vi "detect connected chassis.vi"(8 "error in":errorcluster, 11 "system session in":refnum<k21>) -> (0 "error out":errorcluster, 2 "chassis":T2 {"remote chassis"."product ID" format="%.0x"; "local chassis"."product ID" format="%.0x"}, 3 "system session out":refnum<k21>)   [LabVIEW 2014, in "SMI.lvlib" / "Controller.lvclass"]
uses:
  Controller.lvclass
  Chassis/chassis information.ctl
  <vilib>/nisyscfg/Close (System).vi
  <vilib>/nisyscfg/Close (Filter).vi
  <vilib>/nisyscfg/Close (Resources).vi
  <vilib>/regexp/Match Regular Expression.xnode
  <resource>/objmgr/niflexriosae.rc
  <vilib>/nisyscfg/nisyscfg.lvlib
  <resource>/objmgr/nisysapi.rc
  Chassis/Chassis.lvclass
  SMI.lvlib
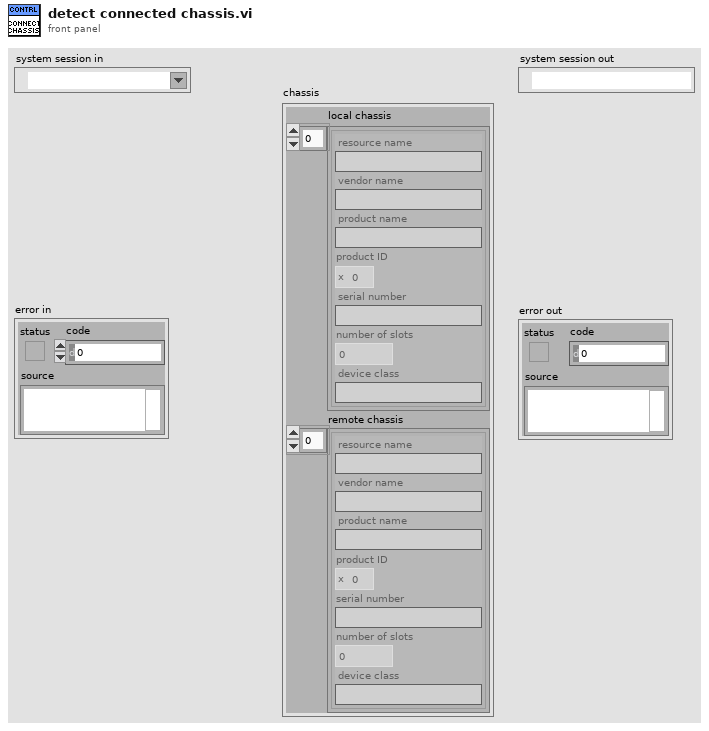
[diagram p1: front panel]
types:
  T1 = typedef "SMI.lvlib/Chassis.lvclass/chassis information.ctl" = cluster{"resource name":string, "vendor name":string, "product name":string, "product ID":u16, "serial number":string, "number of slots":i32, "device class":string}
  T2 = cluster{"local chassis":T1[], "remote chassis":T1[]}
  T3 = cluster{"Local Chassis":T1[], "Remote Chassis":T1[]}
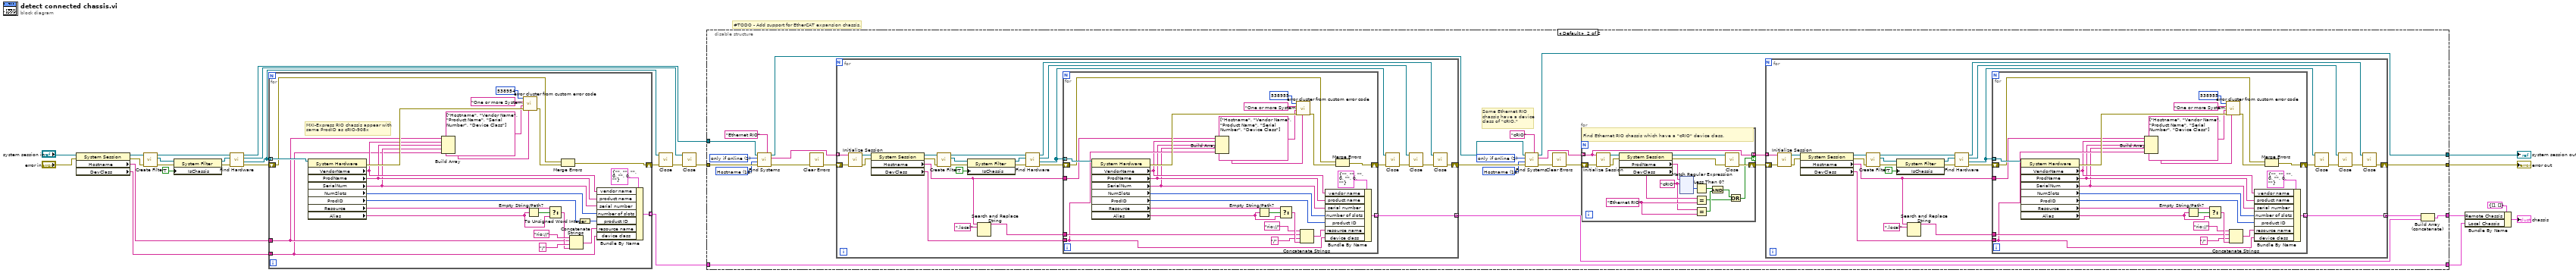
[diagram p0: block diagram]
diagram:
  # "#TODO - Add support for EtherCAT expansion chassis."
  n1 = property class="System Session"(reference="system session in", error in="error in") -> (reference out=w8:refnum<k21>, error out=w7:errorcluster, "Hostname"=w6:string, "DevClass"=w1:string)
  n2 = call <vilib>:"Create Filter.vi"("error in (no error)"=w7, "Session in"=w8) -> ("error out"=w5:errorcluster, "Filter out"=w4:refnum<k20>, "Session out"=w18:refnum<k21>)  [unwired: 7 in]
  n3 = property class="System Filter"(reference=w4, error in=w5, "IsChassis"=TRUE ("Is Chassis")) -> (reference out=w17:refnum<k20>, error out=w16:errorcluster)
  n4 = call <vilib>:"Find Hardware.vi"("error in (no error)"=w16, "Filter in"=w17, "Session in"=w18) -> ("error out"=w15:errorcluster, "Resources out"=w12:refnum<k20>[], "Filter out"=w11:refnum<k20>, "Session out"=w9:refnum<k21>)  [unwired: 5 in]
  n5 = for {
    tunnel: w12 -> [w52] mode=indexing
    shift-right: [w31] -> w13
    shift-left: w15 -> [w33]
    tunnel: [w51] -> w2 mode=indexing
    tunnel: w6 -> [w38]
    tunnel: w1 -> [w34]
    # "MXI-Express RIO chassis appear with\nsame ProdID as cRIO-908x"
    n6 = property class="System Hardware"(reference=w52) -> (error out=w39:errorcluster, "VendorName"=w37:string, "ProdName"=w36:string, "SerialNum"=w35:string, "NumSlots"=w50:i32, "ProdID"=w40:u32, "Resource"=w44:string, "Alias"=w45:string)  [unwired: 1 in, 1 out]
    n7 = Build Array(w38, w37, w36, w35, w34) -> (w29:string[])
    n8 = call "error cluster from custom error code.vi"("string values"=w29, "error in"=w39, "keys"=string[] ["Hostname", "Vendor Name", "Product Name", "Serial Number", "Device Class"], "error message"="One or more System Hardware properties are not available for the target chassis.", "custom error code (0)"=538954 ("error code (0)")) -> ("error out"=w32:errorcluster)  [unwired: 6 in]
    n9 = Empty String/Path?(string/path=w45) -> (empty?=w46:bool)
    n10 = Select(t=w44, s=w46, f=w45) -> (s? t:f=w43:string)
    n11 = Merge Errors(w33, w32) -> (w31:errorcluster)
    n12 = Concatenate Strings("rio://" ("string"), w38, "/" ("string"), w43) -> (w49:string)
    n13 = To Unsigned Word Integer(number=w40) -> (unsigned 16bit integer=w41:u16)
    n14 = Bundle By Name(cluster=T1 {"resource name"="", "vendor name"="", "product name"="", "product ID"=0, "serial number"="", "number of slots"=0, "device class"=""} ("Chassis Information"), "vendor name"=w37, "product name"=w36, "serial number"=w35, "number of slots"=w50, "product ID"=w41, "resource name"=w49, "device class"=w34) -> (w51:T1)
  }
  n15 = call-poly <vilib>:"Close.vi"("error in (no error)"=w13, "Resources in"=w12) -> ("error out"=w14:errorcluster)  [unwired: 9 in]
  n16 = call-poly <vilib>:"Close.vi"("error in (no error)"=w14, "Filter in"=w11) -> ("error out"=w10:errorcluster)  [unwired: 9 in]
  n17 = disable-structure shown="Default" {
    disable-tunnel: w2 -> [w53 w71]
    disable-tunnel: w10 -> [w55 w79]
    disable-tunnel: w9 -> [w54 w78]
    disable-tunnel: [w55 w68] -> w26
    disable-tunnel: [_ w56] -> w21
    disable-tunnel: [w54 w67] -> w23
    disable-tunnel: [w53 w71] -> w20
    frame condition #0 {
      # "Possible CAR: PharLap and VxWorks targets cannot detect Ethernet RIO chassis using Find Systems.vi."
    }
    frame condition #1 (active) {
      w64 = u32 1 items=["none"=0, "only if online"=1, "all"=3] ("Include Cached Results (all)")
      w63 = u32 16 items=["Hostname"=16, "Hostname (IP)"=18, "Hostname (MAC)"=19, "IP"=32, "IP (Hostname)"=33, "IP (MAC)"=35, "MAC"=48, "MAC (Hostname)"=49, "MAC (IP)"=50] ("Output (Hostname and IP)")
      w75 = u32 1 items=["none"=0, "only if online"=1, "all"=3] ("Include Cached Results (all)")
      w76 = u32 16 items=["Hostname"=16, "Hostname (IP)"=18, "Hostname (MAC)"=19, "IP"=32, "IP (Hostname)"=33, "IP (MAC)"=35, "MAC"=48, "MAC (Hostname)"=49, "MAC (IP)"=50] ("Output (Hostname and IP)")
      # "Some Ethernet RIO\nchassis have a device \nclass of \"cRIO.\""
      n18 = call <vilib>:"Find Systems.vi"("Device Class"="Ethernet RIO", "error in (no error)"=w79, "Output (Hostname and IP)"=w76, "Include Cached Results (all)"=w75, "Session in (localhost)"=w78) -> ("error out"=w72:errorcluster, "Detected Systems"=w77:string[], "Session out"=w70:refnum<k21>)  [unwired: 4 in]
      n19 = call <vilib>:"Clear Errors.vi"("error in (no error)"=w72) -> ("error out"=w73:errorcluster)  [unwired: 5 in, 1 out]
      n20 = for {
        shift-right: [w275] -> w69
        shift-left: w73 -> [w286]
        tunnel: [w277] -> w57 mode=concatenating
        tunnel: w77 -> [w273] mode=indexing
        n21 = call <vilib>:"Initialize Session.vi"("error in (no error)"=w286, "Target (localhost)"=w273) -> ("error out"=w270:errorcluster, "Session out"=w272:refnum<k21>)  [unwired: 8 in]
        n22 = property class="System Session"(reference=w272, error in=w270) -> (reference out=w271:refnum<k21>, error out=w269:errorcluster, "Hostname"=w262:string, "DevClass"=w263:string)
        n23 = call <vilib>:"Create Filter.vi"("error in (no error)"=w269, "Session in"=w271) -> ("error out"=w264:errorcluster, "Filter out"=w265:refnum<k20>, "Session out"=w278:refnum<k21>)  [unwired: 7 in]
        n24 = property class="System Filter"(reference=w265, error in=w264, "IsChassis"=TRUE ("Is Chassis")) -> (reference out=w279:refnum<k20>, error out=w280:errorcluster)
        n25 = Search and Replace String(input string=w262, search string=".local") -> (result string=w268:string)  [unwired: 6 in, 3 out]
        n26 = call <vilib>:"Find Hardware.vi"("error in (no error)"=w280, "Filter in"=w279, "Session in"=w278) -> ("error out"=w281:errorcluster, "Resources out"=w284:refnum<k20>[], "Filter out"=w285:refnum<k20>, "Session out"=w276:refnum<k21>)  [unwired: 5 in]
        n27 = for {
          tunnel: w284 -> [w312] mode=indexing
          shift-right: [w296] -> w283
          shift-left: w281 -> [w298]
          tunnel: [w311] -> w277 mode=indexing
          tunnel: w268 -> [w301]
          tunnel: w263 -> [w294]
          tunnel: w262 -> [w295]
          n28 = property class="System Hardware"(reference=w312) -> (error out=w299:errorcluster, "VendorName"=w293:string, "ProdName"=w292:string, "SerialNum"=w291:string, "NumSlots"=w310:i32, "ProdID"=w309:u32, "Resource"=w303:string, "Alias"=w302:string)  [unwired: 1 in, 1 out]
          n29 = Build Array(w295, w293, w292, w291, w294) -> (w288:string[])
          n30 = Empty String/Path?(string/path=w302) -> (empty?=w307:bool)
          n31 = Select(t=w303, s=w307, f=w302) -> (s? t:f=w308:string)
          n32 = call "error cluster from custom error code.vi"("string values"=w288, "error in"=w299, "keys"=string[] ["Hostname", "Vendor Name", "Product Name", "Serial Number", "Device Class"], "error message"="One or more System Hardware properties are not available for the Ethernet RIO remote chassis.", "custom error code (0)"=538955 ("error code (0)")) -> ("error out"=w297:errorcluster)  [unwired: 6 in]
          n33 = Concatenate Strings("rio://" ("string"), w301, "/" ("string"), w308) -> (w304:string)
          n34 = Bundle By Name(cluster=T1 {"resource name"="", "vendor name"="", "product name"="", "product ID"=0, "serial number"="", "number of slots"=0, "device class"=""} ("Chassis Information"), "vendor name"=w293, "product name"=w292, "serial number"=w291, "number of slots"=w310, "product ID"=w309, "resource name"=w304, "device class"=w294) -> (w311:T1)
          n35 = Merge Errors(w298, w297) -> (w296:errorcluster)
        }
        n36 = call-poly <vilib>:"Close.vi"("error in (no error)"=w283, "Resources in"=w284) -> ("error out"=w282:errorcluster)  [unwired: 9 in]
        n37 = call-poly <vilib>:"Close.vi"("error in (no error)"=w282, "Filter in"=w285) -> ("error out"=w274:errorcluster)  [unwired: 9 in]
        n38 = call-poly <vilib>:"Close.vi"("error in (no error)"=w274, "Session in"=w276) -> ("error out"=w275:errorcluster)  [unwired: 9 in]
      }
      n39 = call <vilib>:"Find Systems.vi"("Device Class"="cRIO", "error in (no error)"=w69, "Output (Hostname and IP)"=w63, "Include Cached Results (all)"=w64, "Session in (localhost)"=w70) -> ("error out"=w66:errorcluster, "Detected Systems"=w62:string[], "Session out"=w67:refnum<k21>)  [unwired: 4 in]
      n40 = call <vilib>:"Clear Errors.vi"("error in (no error)"=w66) -> ("error out"=w61:errorcluster)  [unwired: 5 in, 1 out]
      n41 = for {
        tunnel: w62 -> [w94] mode=indexing
        tunnel: [w94] -> w59 mode=indexing if=w80
        shift-right: [w91] -> w60
        shift-left: w61 -> [w93]
        w86 = "cRIO" ("regular expression")
        w89 = "Ethernet RIO" ("y")
        # "Find Ethernet RIO chassis which have a \"cRIO\" device class."
        n42 = call <vilib>:"Initialize Session.vi"("error in (no error)"=w93, "Target (localhost)"=w94) -> ("error out"=w96:errorcluster, "Session out"=w95:refnum<k21>)  [unwired: 8 in]
        n43 = property class="System Session"(reference=w95, error in=w96) -> (reference out=w90:refnum<k21>, error out=w92:errorcluster, "ProdName"=w81:string, "DevClass"=w88:string)
        n44 = xnode "Match Regular Expression"("input string"=w81, "regular expression"=w86) -> ("offset past match"=w87:i32)  [unwired: 4 in, 4 out]
        n45 = Less Than 0?(x=w87) -> (x < 0?=w85:bool)
        n46 = Equal?(x=w88, y=w89) -> (x = y?=w82:bool)
        n47 = Equal?(x=w86, y=w89) -> (x = y?=w84:bool)
        n48 = And(x=w85, y=w84) -> (x .and. y?=w83:bool)
        n49 = call-poly <vilib>:"Close.vi"("error in (no error)"=w92, "Session in"=w90) -> ("error out"=w91:errorcluster)  [unwired: 9 in]
        n50 = Or(x=w83, y=w82) -> (x .or. y?=w80:bool)
      }
      n51 = for {
        shift-right: [w224] -> w68
        shift-left: w60 -> [w235]
        tunnel: [w226] -> w58 mode=concatenating
        tunnel: w59 -> [w222] mode=indexing
        n52 = call <vilib>:"Initialize Session.vi"("error in (no error)"=w235, "Target (localhost)"=w222) -> ("error out"=w219:errorcluster, "Session out"=w221:refnum<k21>)  [unwired: 8 in]
        n53 = property class="System Session"(reference=w221, error in=w219) -> (reference out=w220:refnum<k21>, error out=w218:errorcluster, "Hostname"=w211:string, "DevClass"=w212:string)
        n54 = call <vilib>:"Create Filter.vi"("error in (no error)"=w218, "Session in"=w220) -> ("error out"=w213:errorcluster, "Filter out"=w214:refnum<k20>, "Session out"=w227:refnum<k21>)  [unwired: 7 in]
        n55 = property class="System Filter"(reference=w214, error in=w213, "IsChassis"=TRUE ("Is Chassis")) -> (reference out=w228:refnum<k20>, error out=w229:errorcluster)
        n56 = Search and Replace String(input string=w211, search string=".local") -> (result string=w217:string)  [unwired: 6 in, 3 out]
        n57 = call <vilib>:"Find Hardware.vi"("error in (no error)"=w229, "Filter in"=w228, "Session in"=w227) -> ("error out"=w230:errorcluster, "Resources out"=w233:refnum<k20>[], "Filter out"=w234:refnum<k20>, "Session out"=w225:refnum<k21>)  [unwired: 5 in]
        n58 = for {
          tunnel: w233 -> [w261] mode=indexing
          shift-right: [w245] -> w232
          shift-left: w230 -> [w247]
          tunnel: [w260] -> w226 mode=indexing
          tunnel: w217 -> [w250]
          tunnel: w212 -> [w243]
          tunnel: w211 -> [w244]
          n59 = property class="System Hardware"(reference=w261) -> (error out=w248:errorcluster, "VendorName"=w242:string, "ProdName"=w241:string, "SerialNum"=w240:string, "NumSlots"=w259:i32, "ProdID"=w258:u32, "Resource"=w252:string, "Alias"=w251:string)  [unwired: 1 in, 1 out]
          n60 = Build Array(w244, w242, w241, w240, w243) -> (w237:string[])
          n61 = Empty String/Path?(string/path=w251) -> (empty?=w256:bool)
          n62 = Select(t=w252, s=w256, f=w251) -> (s? t:f=w257:string)
          n63 = call "error cluster from custom error code.vi"("string values"=w237, "error in"=w248, "keys"=string[] ["Hostname", "Vendor Name", "Product Name", "Serial Number", "Device Class"], "error message"="One or more System Hardware properties are not available for the Ethernet RIO remote chassis.", "custom error code (0)"=538955 ("error code (0)")) -> ("error out"=w246:errorcluster)  [unwired: 6 in]
          n64 = Concatenate Strings("rio://" ("string"), w250, "/" ("string"), w257) -> (w253:string)
          n65 = Bundle By Name(cluster=T1 {"resource name"="", "vendor name"="", "product name"="", "product ID"=0, "serial number"="", "number of slots"=0, "device class"=""} ("Chassis Information"), "vendor name"=w242, "product name"=w241, "serial number"=w240, "number of slots"=w259, "product ID"=w258, "resource name"=w253, "device class"=w243) -> (w260:T1)
          n66 = Merge Errors(w247, w246) -> (w245:errorcluster)
        }
        n67 = call-poly <vilib>:"Close.vi"("error in (no error)"=w232, "Resources in"=w233) -> ("error out"=w231:errorcluster)  [unwired: 9 in]
        n68 = call-poly <vilib>:"Close.vi"("error in (no error)"=w231, "Filter in"=w234) -> ("error out"=w223:errorcluster)  [unwired: 9 in]
        n69 = call-poly <vilib>:"Close.vi"("error in (no error)"=w223, "Session in"=w225) -> ("error out"=w224:errorcluster)  [unwired: 9 in]
      }
      n70 = Build Array (concatenate)(w58, w57) -> (w56:T1[])
    }
  }
  "error out" <- w26
  "system session out" <- w23
  n71 = Bundle By Name(cluster=T3 {"Local Chassis"=[], "Remote Chassis"=[]} ("Chassis"), "Remote Chassis"=w21, "Local Chassis"=w20) -> (→"chassis":T3)
